vi "Mutate Multi FPGA.vi"(8 "error in (no error)":errorcluster, 11 "Device Ref in":T1 format="%.0x") -> (0 "error out":errorcluster, 3 "Device Ref out":T1 format="%.0x")   [LabVIEW 2020, in "Engine Simulation Toolkit System Explorer.lvlib"]
uses:
  Engine Simulation Toolkit System Explorer.lvlib
  <vilib>/NI VeriStand/Custom Device API/Custom Device Item Ref.ctl
  Shared/Channel.ctl
  <vilib>/NI VeriStand/Custom Device API/Custom Device Channel Type.ctl
  Shared/Properties.vi
  Shared/Constants and GUIDs.vi
  <vilib>/NI VeriStand/Custom Device API/Get Item Property (Boolean).vi
  <vilib>/NI VeriStand/Custom Device API/Get Item Property (String).vi
  <vilib>/NI VeriStand/Custom Device API/Set Item Property (String Array).vi
  <vilib>/NI VeriStand/Custom Device API/Get Item Property (Dependent File).vi
  <vilib>/NI VeriStand/Custom Device API/Set Item Property (String).vi
  <vilib>/NI VeriStand/Custom Device Tools/Custom Device Utility Library/NI VeriStand - Search for All Items by GUID.vi
  Shared/Engine Simulation Toolkit Shared.lvlib
  <vilib>/NI VeriStand/Custom Device API/Custom Device API.lvlib
  <vilib>/NI VeriStand/Custom Device Tools/Custom Device Utility Library/Custom Device Utility Library.lvlib
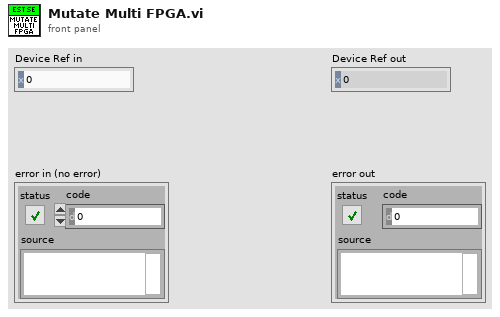
[diagram p1: front panel]
types:
  T1 = typedef "Custom Device API.lvlib/Custom Device Item Ref.ctl" = u64
  T2 = typedef "Engine Simulation Toolkit Shared.lvlib/Channel.ctl" = cluster{"Name":string, "Units":string, "Default":dbl, "Description":string, "Scalable":bool}
  T3 = typedef "Custom Device API.lvlib/Custom Device Channel Type.ctl" = enum16{"Input", "Output"}
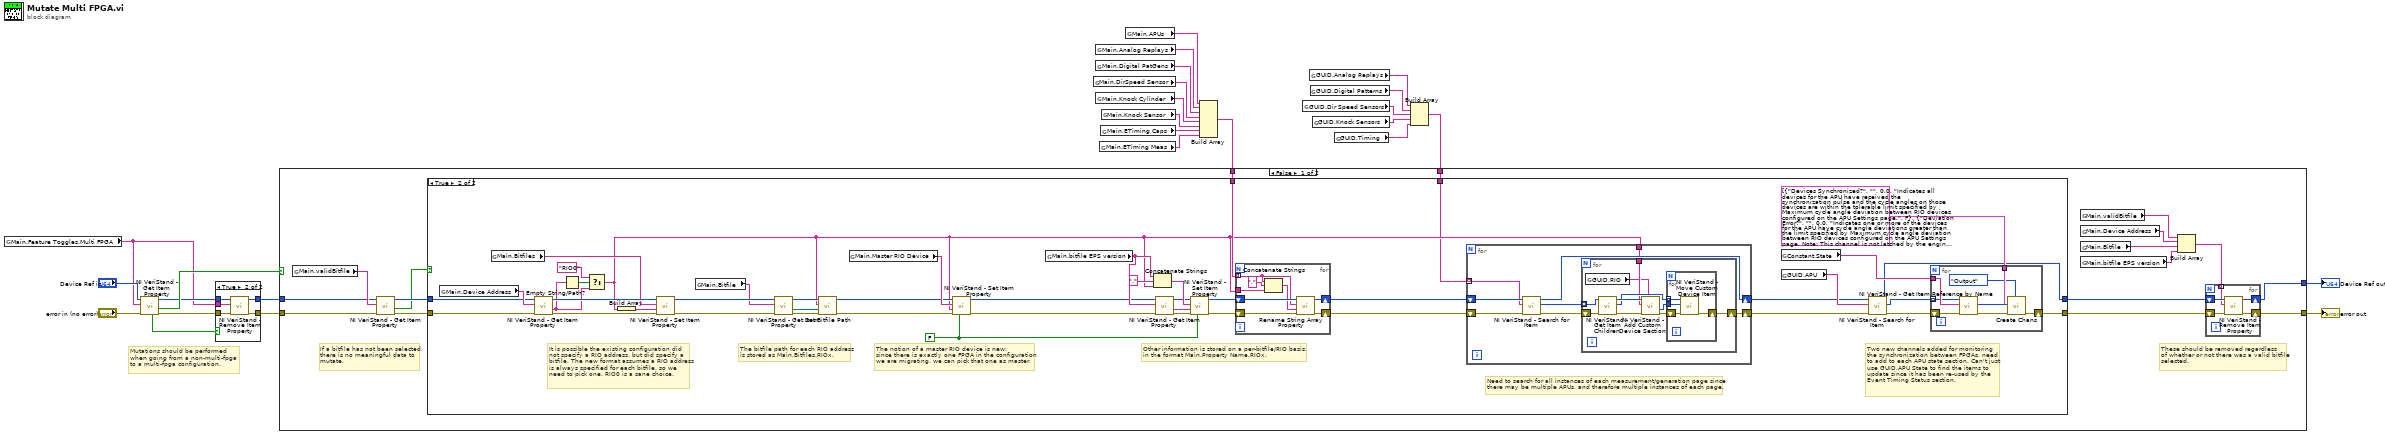
[diagram p0: block diagram]
diagram:
  # "Mutations should be performed\nwhen going from a non-multi-fpga\nto a multi-fpga configuration."
  n1 = global read "Properties.vi" "Main.Feature Toggles.Multi FPGA"() -> (w2:string)
  n2 = call-poly <vilib>:"NI VeriStand - Get Item Property.vi"("error in (no error)"="error in (no error)", "Property Name"=w2, "Item Ref in"="Device Ref in") -> ("error out"=w6:errorcluster, "Value"=w9:bool, "Item Ref out"=w5:T1, "Found?"=w1:bool)  [unwired: 5 in]
  n3 = case shown="True" w1 {
    tunnel: w6 -> [w27 w33]
    tunnel: w5 -> [w28 w32]
    tunnel: [w27 w31] -> w4
    tunnel: [w28 w30] -> w3
    tunnel: w2 -> [_ w29]
    frame False {
    }
    frame True {
      n4 = call <vilib>:"NI VeriStand - Remove Item Property.vi"("error in (no error)"=w33, "Property Name"=w29, "Item Ref in"=w32) -> ("error out"=w31:errorcluster, "Item Ref out"=w30:T1)  [unwired: 6 in, 1 out]
    }
  }
  n5 = global read "Properties.vi" "Main.DirSpeed Sensor"() -> (w22:string)
  n6 = global read "Properties.vi" "Main.Analog Replays"() -> (w20:string)
  n7 = global read "Properties.vi" "Main.Digital PatGens"() -> (w21:string)
  n8 = global read "Properties.vi" "Main.Knock Cylinder"() -> (w23:string)
  n9 = global read "Properties.vi" "Main.ETiming Meas"() -> (w25:string)
  n10 = global read "Properties.vi" "Main.ETiming Caps"() -> (w24:string)
  n11 = global read "Properties.vi" "Main.Knock Sensor"() -> (w26:string)
  n12 = global read "Properties.vi" "Main.APUs"() -> (w19:string)
  n13 = Build Array(w19, w20, w21, w22, w23, w26, w24, w25) -> (w18:string[])
  n14 = global read "Constants and GUIDs.vi" "GUID.Dir Speed Sensors"() -> (w15:string)
  n15 = global read "Constants and GUIDs.vi" "GUID.Analog Replays"() -> (w13:string)
  n16 = global read "Constants and GUIDs.vi" "GUID.Digital Patterns"() -> (w14:string)
  n17 = global read "Constants and GUIDs.vi" "GUID.Knock Sensors"() -> (w16:string)
  n18 = global read "Constants and GUIDs.vi" "GUID.Timing"() -> (w17:string)
  n19 = Build Array(w13, w14, w15, w16, w17) -> (w12:string[])
  n20 = case shown="False" w9 {
    tunnel: w18 -> [w50 _]
    tunnel: w4 -> [w48 w141]
    tunnel: w12 -> [w45 _]
    tunnel: [w35 w141] -> w10
    tunnel: [w36 w140] -> w11
    tunnel: w3 -> [w34 w140]
    frame False {
      # "These should be removed regardless\nof whether or not there was a valid bitfile\nselected."
      # "If a bitfile has not been selected,\nthere is no meaningful data to\nmutate."
      n21 = global read "Properties.vi" "Main.validBitfile"() -> (w49:string)
      n22 = call-poly <vilib>:"NI VeriStand - Get Item Property.vi"("error in (no error)"=w48, "Property Name"=w49, "Item Ref in"=w34) -> ("error out"=w47:errorcluster, "Value"=w44:bool, "Item Ref out"=w46:T1)  [unwired: 5 in, 1 out]
      n23 = case shown="True" w44 {
        tunnel: w47 -> [w51 w54]
        tunnel: w46 -> [w52 w53]
        tunnel: [w52 w55] -> w42
        tunnel: [w51 w62] -> w43
        tunnel: w50 -> [_ w79]
        tunnel: w45 -> [_ w64]
        frame False {
        }
        frame True {
          w68 = FALSE ("Binary String (T)")
          # "Two new channels added for monitoring\nthe synchronization between FPGAs, need\nto add to each APU state section. Can't just\nuse GUID.APU State to find the items to\nupdate since it has been re-used by the \nEvent Timing Status section."
          # "Need to search for all instances of each measurement/generation page since\nthere may be multiple APUs, and therefore multiple instances of each page."
          # "Other information is stored on a per-bitfile/RIO basis,\nin the format Main.Property Name.RIOx."
          # "The notion of a master RIO device is new;\nsince there is exactly one FPGA in the configuration\nwe are migrating, we can pick that one as master."
          # "The bitfile path for each RIO address\nis stored as Main.Bitfiles.RIOx."
          # "It is possible the existing configuration did\nnot specify a RIO address, but did specify a\nbitfile. The new format assumes a RIO address\nis always specified for each bitfile, so we\nneed to pick one. RIO0 is a sane choice."
          n24 = global read "Properties.vi" "Main.Device Address"() -> (w88:string)
          n25 = global read "Properties.vi" "Main.Bitfiles"() -> (w80:string)
          n26 = call-poly <vilib>:"NI VeriStand - Get Item Property.vi"("error in (no error)"=w54, "Property Name"=w88, "Item Ref in"=w53) -> ("error out"=w94:errorcluster, "Value"=w77:string, "Item Ref out"=w95:T1)  [unwired: 5 in, 1 out]
          n27 = Empty String/Path?(string/path=w77) -> (empty?=w78:bool)
          n28 = Select(t="RIO0", s=w78, f=w77) -> (s? t:f=w67:string)
          n29 = Build Array(w67) -> (w96:string[])
          n30 = call-poly <vilib>:"NI VeriStand - Set Item Property.vi"("error in (no error)"=w94, "Value"=w96, "Property Name"=w80, "Item Ref in"=w95) -> ("error out"=w89:errorcluster, "Item Ref out"=w90:T1)  [unwired: 5 in, 1 out]
          n31 = global read "Properties.vi" "Main.Bitfile"() -> (w87:string)
          n32 = call-poly <vilib>:"NI VeriStand - Get Item Property.vi"("error in (no error)"=w89, "Property Name"=w87, "Item Ref in"=w90) -> ("error out"=w93:errorcluster, "Path"=w92:path, "Item Ref out"=w91:T1)  [unwired: 4 in, 2 out]
          n33 = call "Set Bitfile Path.vi"("error in (no error)"=w93, "Bitfile Path in"=w92, "RIO Device Address in"=w67, "Item Ref in"=w91) -> ("error out"=w71:errorcluster, "Item Ref out"=w70:T1)  [unwired: 6 in]
          n34 = global read "Properties.vi" "Main.Master RIO Device"() -> (w73:string)
          n35 = call-poly <vilib>:"NI VeriStand - Set Item Property.vi"("Binary String (T)"=w68, "error in (no error)"=w71, "Value"=w67, "Property Name"=w73, "Item Ref in"=w70) -> ("error out"=w72:errorcluster, "Item Ref out"=w69:T1)  [unwired: 4 in, 1 out]
          n36 = global read "Properties.vi" "Main.bitfile EPS version"() -> (w82:string)
          n37 = Concatenate Strings(w82, "." ("string"), w67) -> (w83:string)
          n38 = call-poly <vilib>:"NI VeriStand - Get Item Property.vi"("error in (no error)"=w72, "Property Name"=w82, "Item Ref in"=w69) -> ("error out"=w85:errorcluster, "Value"=w84:string, "Item Ref out"=w81:T1)  [unwired: 5 in, 1 out]
          n39 = call-poly <vilib>:"NI VeriStand - Set Item Property.vi"("Binary String (T)"=w68, "error in (no error)"=w85, "Value"=w84, "Property Name"=w83, "Item Ref in"=w81) -> ("error out"=w75:errorcluster, "Item Ref out"=w74:T1)  [unwired: 4 in, 1 out]
          n40 = for {
            tunnel: w67 -> [w133]
            tunnel: w79 -> [w130] mode=indexing
            shift-right: [w128] -> w65
            shift-left: w75 -> [w132]
            shift-right: [w127] -> w66
            shift-left: w74 -> [w131]
            n41 = Concatenate Strings(w130, "." ("string"), w133) -> (w129:string)
            n42 = call "Rename String Array Property.vi"("error in (no error)"=w132, "New Name"=w129, "Old Name"=w130, "Item Ref in"=w131) -> ("error out"=w128:errorcluster, "Item Ref out"=w127:T1)  [unwired: 6 in]
          }
          n43 = for {
            tunnel: w67 -> [w105]
            shift-right: [w108] -> w57
            shift-left: w65 -> [w109]
            shift-right: [w107] -> w58
            shift-left: w66 -> [w110]
            tunnel: w64 -> [w106] mode=indexing
            n44 = call-poly <vilib>:"NI VeriStand - Search for Item.vi"("error in"=w109, "Item GUID"=w106, "Section Ref in"=w110) -> ("error out"=w111:errorcluster, "Item Refs"=w112:T1[], "Section Ref out"=w107:T1)  [unwired: 5 in, 1 out]
            n45 = for {
              tunnel: w112 -> [w122] mode=indexing
              tunnel: w105 -> [w115]
              shift-right: [w113] -> w108
              shift-left: w111 -> [w119]
              n46 = global read "Constants and GUIDs.vi" "GUID.RIO"() -> (w114:string)
              n47 = call <vilib>:"NI VeriStand - Get Item Children.vi"("error in (no error)"=w119, "Item Ref in"=w122) -> ("error out"=w121:errorcluster, "Child Refs"=w116:T1[], "Item Ref out"=w120:T1)  [unwired: 6 in, 1 out]
              n48 = call <vilib>:"NI VeriStand - Add Custom Device Section.vi"("GUID (Default Section)"=w114, "error in (no error)"=w121, "Section Name"=w115, "Parent Ref in"=w120) -> ("error out"=w117:errorcluster, "Section Ptr"=w118:T1)  [unwired: 4 in, 2 out]
              n49 = for {
                tunnel: w118 -> [w126]
                tunnel: w116 -> [w124] mode=indexing
                shift-right: [w123] -> w113
                shift-left: w117 -> [w125]
                n50 = call <vilib>:"NI VeriStand - Move Custom Device Item.vi"("error in (no error)"=w125, "New Parent Ref in"=w126, "Item Ref in"=w124) -> ("error out"=w123:errorcluster)  [unwired: 6 in, 2 out]
              }
            }
          }
          n51 = global read "Constants and GUIDs.vi" "Constant.State"() -> (w63:string)
          n52 = global read "Constants and GUIDs.vi" "GUID.APU"() -> (w59:string)
          n53 = call-poly <vilib>:"NI VeriStand - Search for Item.vi"("error in"=w57, "Item GUID"=w59, "Section Ref in"=w58) -> ("error out"=w60:errorcluster, "Item Refs"=w56:T1[], "Section Ref out"=w55:T1)  [unwired: 5 in, 1 out]
          n54 = for {
            tunnel: w63 -> [w104]
            tunnel: T2[] [{"Name"="Devices Synchronized?", "Units"="", "Default"=0.0, "Description"="Indicates all devices for the APU have received the synchronization pulse and the cycle angles on those devices are within the tolerable limit specified by Maximum cycle angle deviation between RIO devices configured on the APU Settings page.", "Scalable"=FALSE}, {"Name"="Deviation Error?", "Units"="", "Default"=0.0, "Description"="Indicates one or more of the devices for the APU have cycle angle deviations greater than the limit specified by Maximum cycle angle deviation between RIO devices configured on the APU Settings page. Note: This channel is not latched by the engine. It is updated each iteration of the PCL. If your test needs to error/stop when this channel is true, you must implement some sort of latch in the test execution.", "Scalable"=FALSE}] ("ChanList.APU State") -> [w100]
            tunnel: w56 -> [w97] mode=indexing
            shift-right: [w102] -> w62
            shift-left: w60 -> [w98]
            n55 = call <vilib>:"NI VeriStand - Get Item Reference by Name.vi"("error in (no error)"=w98, "Item Name"=w104, "Parent Ref in"=w97) -> ("error out"=w103:errorcluster, "Item Ref"=w101:T1)  [unwired: 5 in, 2 out]
            n56 = call "Create Chans.vi"("Type"=Custom_Device_Channel_Type."Output", "error in (no error)"=w103, "Channels"=w100, "Section Ptr"=w101) -> ("error out"=w102:errorcluster)  [unwired: 4 in, 3 out]
          }
        }
      }
      n57 = global read "Properties.vi" "Main.validBitfile"() -> (w40:string)
      n58 = global read "Properties.vi" "Main.Device Address"() -> (w41:string)
      n59 = global read "Properties.vi" "Main.Bitfile"() -> (w39:string)
      n60 = global read "Properties.vi" "Main.bitfile EPS version"() -> (w38:string)
      n61 = Build Array(w40, w41, w39, w38) -> (w37:string[])
      n62 = for {
        shift-right: [w136] -> w36
        shift-left: w42 -> [w138]
        tunnel: w37 -> [w135] mode=indexing
        shift-right: [w137] -> w35
        shift-left: w43 -> [w139]
        n63 = call <vilib>:"NI VeriStand - Remove Item Property.vi"("error in (no error)"=w139, "Property Name"=w135, "Item Ref in"=w138) -> ("error out"=w137:errorcluster, "Item Ref out"=w136:T1)  [unwired: 6 in, 1 out]
      }
    }
    frame True {
    }
  }
  "Device Ref out" <- w11
  "error out" <- w10
